vi "KYFG Camera Read Reg.vi"(0 "camHandle":u32, 5 "address":u64, 7 "size":u32, 11 "error in (no error)":errorcluster) -> (4 "camHandle out":u32, 6 "size out":u32, 10 "data out":u8[](array[numeric]), 15 "error out":errorcluster)   [LabVIEW 2023, in "KYFGLib_lv.lvlib"]
doc: "KYFG_API FGSTATUS KYFG_CameraReadReg(CAMHANDLE camHandle, unsigned int address, void* data, unsigned int* size);"
uses:
  KYFGLib_lv.lvlib
  KYFGLib.dll
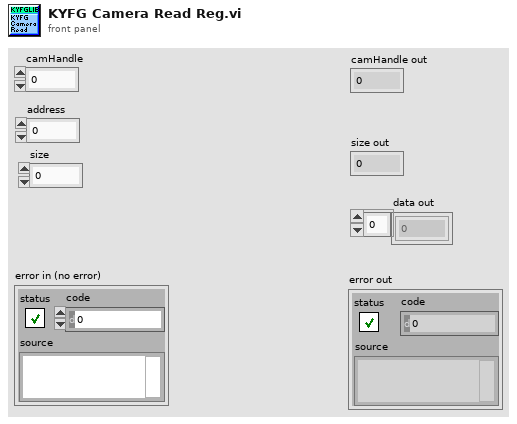
[diagram p1: front panel]
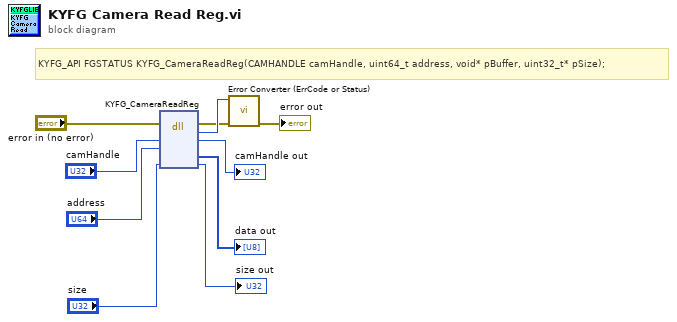
[diagram p0: block diagram]
diagram:
  # "KYFG_API FGSTATUS KYFG_CameraReadReg(CAMHANDLE camHandle, uint64_t address, void* pBuffer, uint32_t* pSize);"
  n1 = dll-call lib="KYFGLib.dll" fn="KYFG_CameraReadReg"(error in="error in (no error)", "camHandle"="camHandle", "address"="address", "pSize"="size") -> (error out=w4:errorcluster, "return type"=w10:u32, "camHandle"=→"camHandle out":u32, "pBuffer"=→"data out":u8[], "pSize"=→"size out":u32)  [unwired: 4 in, 1 out]
  n2 = call "Error Converter (ErrCode or Status).vi"("error in (no error)"=w4, "error code"=w10) -> ("error out"=→"error out":errorcluster)  [unwired: 9 in]
